vi "New XML Document.vi"(8 "error in":errorcluster) -> (0 "error out":errorcluster, 3 "XML Document":refnum<k24>)   [LabVIEW 2026, in "ToastNotification.lvlib" / "Toast Native.lvlib"]
doc: "Create an empty Windows.Data.Xml.Dom.XmlDocument through runtime reflection. Skipped on incoming error. XML Document is acquired and must be closed by the caller, including after later Load XML or display failure. Resolve and release the temporary Type internally. Does not load XML or display a toast."
uses:
  Toast Native.lvlib
  Reflection DotNet/Reflection DotNet.lvlib
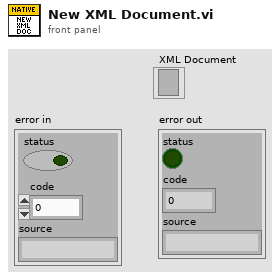
[diagram p1: front panel]
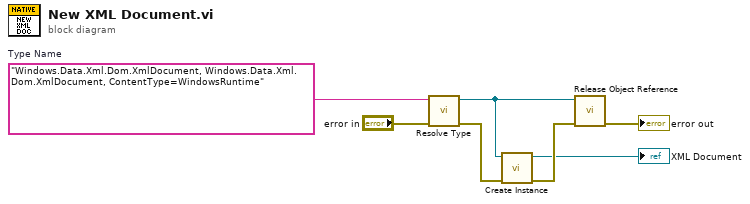
[diagram p0: block diagram]
diagram:
  w4 = "Windows.Data.Xml.Dom.XmlDocument, Windows.Data.Xml.Dom.XmlDocument, ContentType=WindowsRuntime"  # Type Name
  n1 = call "Resolve Type.vi"("error in"="error in", "Type Name"=w4) -> ("error out"=w7:errorcluster, "Runtime Type"=w3:refnum<k24>)  [unwired: 8 in]
  n2 = call "Create Instance.vi"("error in"=w7, "Runtime Type"=w3) -> ("error out"=w6:errorcluster, "Instance"=→"XML Document":refnum<k24>)  [unwired: 8 in]
  n3 = call "Release Object Reference.vi"("error in"=w6, "object"=w3) -> ("error out"=→"error out":errorcluster)  [unwired: 9 in]
